vi "Update Unicode Controls Async.vi"(9 "Stop Event":refnum<user-event>, 10 "Value Change Event":refnum<user-event>, 11 "String Refs":refnum<vi>[](array[refnum])) -> ()   [LabVIEW 2020, in "G-Unicode.lvlib"]
doc: "Update the controls in <b>String Refs</b> with the correct unicode value when a user types text.\n\nAll controls in <b>String Refs</b> will have their Update While Typing? and Force Unicode Text properties set True."
uses:
  G-Unicode.lvlib
  Unicode/Controls/String Encoding.ctl
  Types/UTF-8 String/UTF-8 String.lvclass/UTF-8 String.ctl
  Dialog & User Interface/Polymorphic VIs/Write Control Text/Write String Value (UTF-8 String).vi
  Unicode/Encode String.vi
  Dialog & User Interface/Polymorphic VIs/Write Control Text/Write String Value (UTF-8 String).vi/5206cb6b-04fb-41f5-a37e-29c14f142303.vi
  Conversion/Text to UTF-8.vi
  Conversion/Polymorphic VIs/Text to UTF-8 (LabVIEW String).vi
  Conversion/Encoded UTF-8 String to Encoded UTF-16LE String.vi
  Conversion/UTF-8 to Text.vi
  Conversion/Polymorphic VIs/UTF-8 to Text (LabVIEW String).vi
  Conversion/Encoded UTF-16LE String to Encoded UTF-8 String.vi
  Unicode/Prepend BOM.vi
  Conversion/Text as Encoded String.vi
  Conversion/Polymorphic VIs/Text as Encoded String (UTF-8 String).vi
  Unicode/SubVIs/Byte Order Marks.vi
  Unicode/Detect BOM.vi
  Types/UTF-8 String/Read Encoded UTF-8 String.vi
  Unicode/Detect String Encoding.vi
  User Interface/Write String.vi
  Types/UTF-8 String/UTF-8 String.lvclass
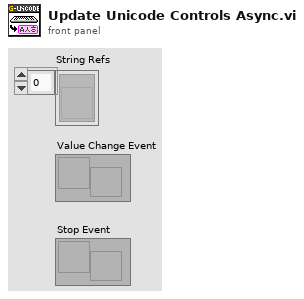
[diagram p1: front panel]
types:
  T1 = typedef "G-Unicode.lvlib/String Encoding.ctl" = enum16{"ANSI", "UTF-8", "UTF-16LE", "UTF-16BE", "Unknown"}
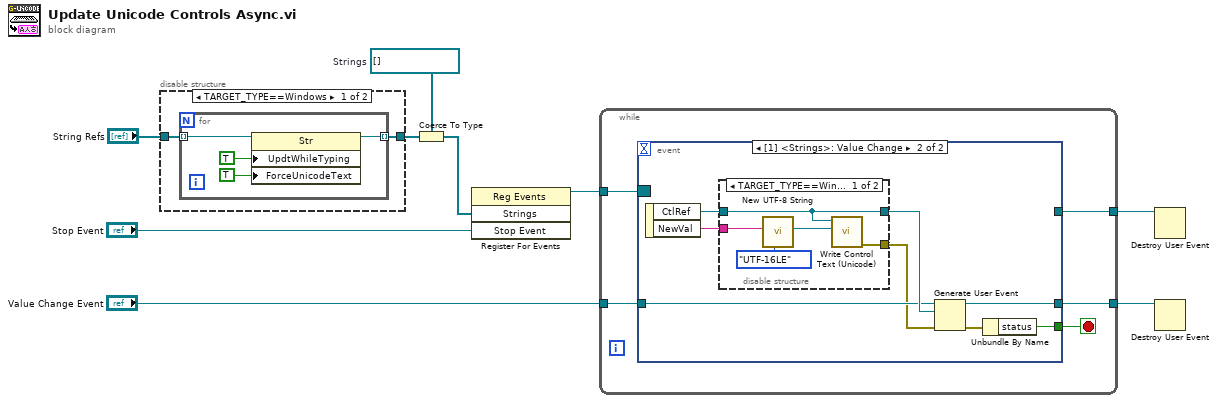
[diagram p0: block diagram]
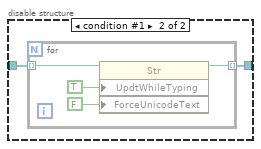
[diagram p2: hidden frame]
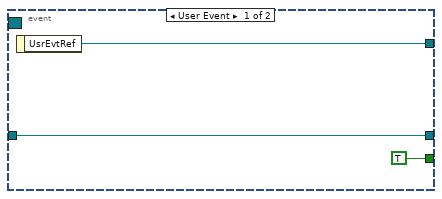
[diagram p3: hidden frame]
diagram:
  w5 = refnum<vi>[] []  # Strings
  n1 = disable-structure shown="TARGET_TYPE==Windows" {
    disable-tunnel: [w11 w17] -> w8
    disable-tunnel: "String Refs" -> [w10 w16]
    frame condition #0 (active) {
      n2 = for {
        tunnel: w10 -> [w12] mode=indexing
        tunnel: [w14] -> w11 mode=indexing
        n3 = property class="Str"(reference=w12, "UpdtWhileTyping"=TRUE ("Update While Typing?"), "ForceUnicodeText"=TRUE ("Force Unicode Text")) -> (reference out=w14:refnum<vi>)  [unwired: 1 in, 1 out]
      }
    }
    frame condition #1 {
      n4 = for {
        tunnel: w16 -> [w19] mode=indexing
        tunnel: [w21] -> w17 mode=indexing
        n5 = property class="Str"(reference=w19, "UpdtWhileTyping"=TRUE ("Update While Typing?"), "ForceUnicodeText"=FALSE ("Force Unicode Text")) -> (reference out=w21:refnum<vi>)  [unwired: 1 in, 1 out]
      }
    }
  }
  n6 = Coerce To Type(0:w8, 1:w5) -> (2:w6:refnum<vi>[])
  n7 = register-events(w6, "Stop Event") -> (reference out=w9:refnum<event-registration>)  [unwired: 2 in, 1 out]
  n8 = while {
    tunnel: w9 -> [w26]
    tunnel: [w24] -> w2
    tunnel: "Value Change Event" -> [w23]
    tunnel: [w22] -> w1
    stop <- w25 stop-if-true
    n9 = event shown="[1] <Strings>: Value Change" {
      selector: w26 -> [_ _]
      dyn-events: _ -> [_ _]
      timeout: _ -> [_ _]
      tunnel: [TRUE w34] -> w25
      tunnel: [w28 w31] -> w24
      tunnel: w23 -> [w28 w32]
      tunnel: [w27 _] -> w22
      event User Event {
        n10 = event-data() -> ("UsrEvtRef"=w27:refnum<user-event>)  [unwired: 1 in]
      }
      event Value Change {
        n11 = event-data() -> ("CtlRef"=w37:refnum<vi>, "NewVal"=w36:string)  [unwired: 1 in]
        n12 = disable-structure shown="TARGET_TYPE==Windows" {
          disable-tunnel: w37 -> [w38 w43]
          disable-tunnel: w36 -> [w42 _]
          disable-tunnel: [w38 w43] -> w33
          disable-tunnel: [w39 _] -> w30
          frame condition #0 (active) {
            n13 = call "New UTF-8 String.vi"("Input Encoding (ANSI)"=String_Encoding."UTF-16LE", "String"=w42) -> ("UTF-8 String"=w40:refnum<class "UTF-8 String.lvclass">)  [unwired: 8 in, 1 out]
            n14 = call-poly "Write Control Text (Unicode).vi"("Value"=w40, "Control Ref"=w38) -> ("error out"=w39:errorcluster)  [unwired: 9 in]
          }
          frame condition #1 {
          }
        }
        n15 = Generate User Event(user event=w32, event data cluster=w33, error in=w30) -> (user event out=w31:refnum<user-event>, error out=w35:errorcluster)  [unwired: 1 in]
        n16 = Unbundle By Name(w35) -> ("status"=w34:bool)
      }
    }
  }
  n17 = Destroy User Event(user event=w1) -> ()  [unwired: 1 in, 1 out]
  n18 = Destroy User Event(user event=w2) -> ()  [unwired: 1 in, 1 out]
